vi "Earth Detection.vi"(8 "error in":errorcluster) -> (0 "error out":errorcluster, 2 "Result":string, 3 "RESULT":bool)   [LabVIEW 2021]
uses:
  DUT/DUT_Cmd.ctl
panel:
  out "number":dbl
  out "Command Response":string
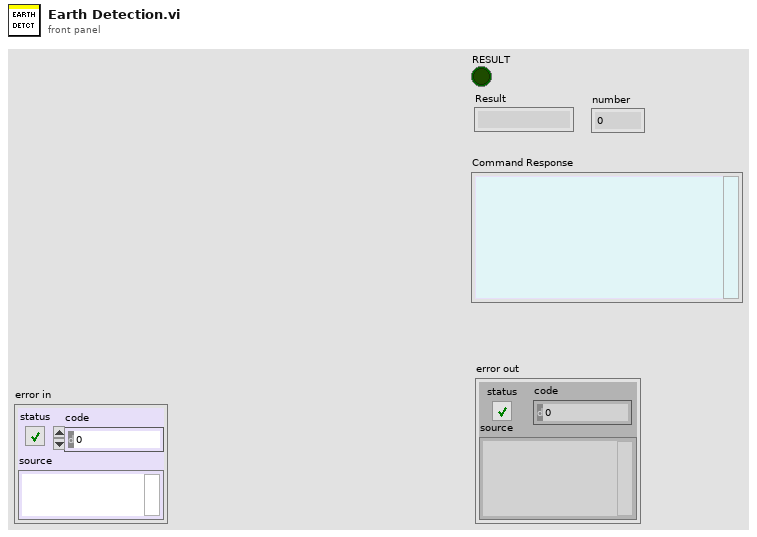
[diagram p1: front panel]
types:
  T1 = typedef "DUT_Cmd.ctl" = enum16{"Unlock serial", "Stop console logs", "Release emergency at start", "Read firmware", "WiFi credentials", "WiFi connected", "WiFi SSID", "Board revision", "ADC_NTC_TEMP", "ADC_TYPE2_RCD_CURRENT", "PCBA serial write", "PCBA serial readback", "Start energy meter", "Energy meter Vac", "Energy meter Iac", "Energy meter PF", "Energy meter energy", "Provision", "Set gateway identity", "CP checklist", "Earth detect", "D+M sense unplugged", "D+M sense plugged", "Output relay weld", "Start diagnostics", "Relay 1 on", "Relay 2 on", "Emergency pressed", "Release emergency", "Emergency released", "Unlock serial for 5 A", "Board current (5 A)", "Unlock serial for 15 A", "Board current (15 A)", "Unlock serial for 0 A", "NFC tag", "Start diagnostics again", "Relay 2 off", "Relay 1 off", "End diagnostics", "Load current (5 A) [No USB station]", "Load current (15 A) [No USB station]", "Load current (0 A) [No USB station]", "NFC tag [No USB station]", "Battery Voltage", "FW Power reset", "Notification LED", "O/P Relay weld Detection", "Earth Detection", "12V ", "5V", "3.3V"}
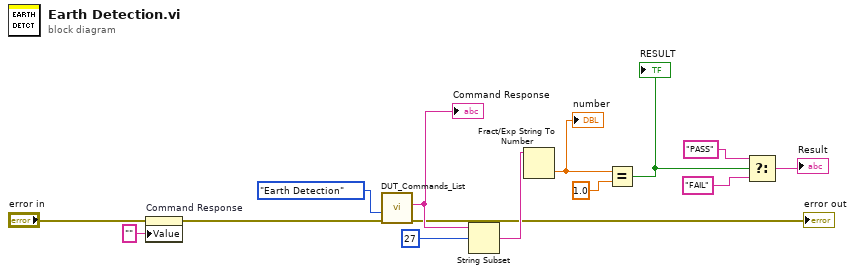
[diagram p0: block diagram]
diagram:
  n1 = property on="Command Response" class="Str"(error in="error in", "Value"="" ("Command Response")) -> (error out=w9:errorcluster)  [unwired: 1 in, 1 out]
  n2 = call "DUT_Commands_List.vi"("error in"=w9, "DUT Cmd"=DUT_Cmd."Earth Detection") -> ("error out"=→"error out":errorcluster, "Command Response"=w7:string)  [unwired: 7 in, 1 out]
  "Command Response" <- w7
  n3 = String Subset(string=w7, offset (0)=27) -> (substring=w5:string)  [unwired: 1 in]
  n4 = Fract/Exp String To Number(string=w5) -> (number=w3:dbl)  [unwired: 3 in, 1 out]
  "number" <- w3
  n5 = Equal?(x=w3, y=1.0 ("lower limit")) -> (x = y?=w2:bool)
  "RESULT" <- w2
  n6 = Select(t="PASS", s=w2, f="FAIL") -> (s? t:f=→"Result":string)
